vi "move2.vi"(8 "error in (no error)":errorcluster caption="错误输入（无错误）", 9 "动效风格":enum16{"风格一", "风格二", "风格三", "风格四"}(ring), 10 "In(T)/Out(F)":bool, 11 "Decor引用句柄":refnum<vi>) -> (0 "error out":errorcluster caption="错误输出")   [LabVIEW 2025, in "XButton.lvlib" / "button3.xctl"]
uses:
  button3.xctl
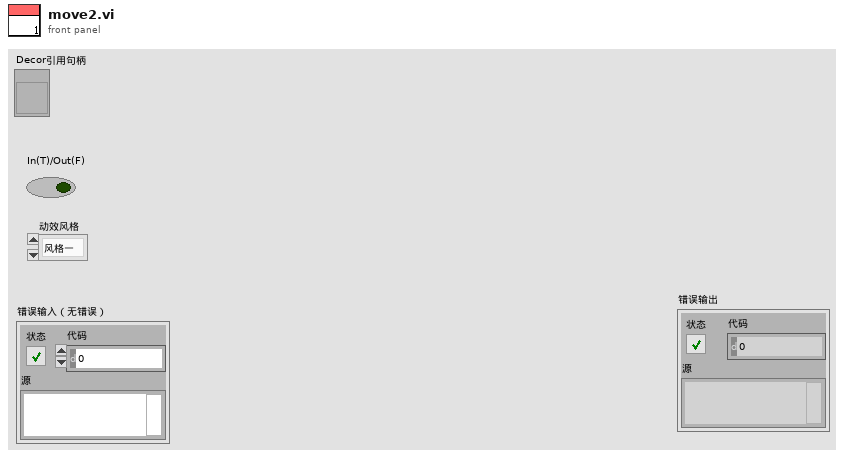
[diagram p1: front panel]
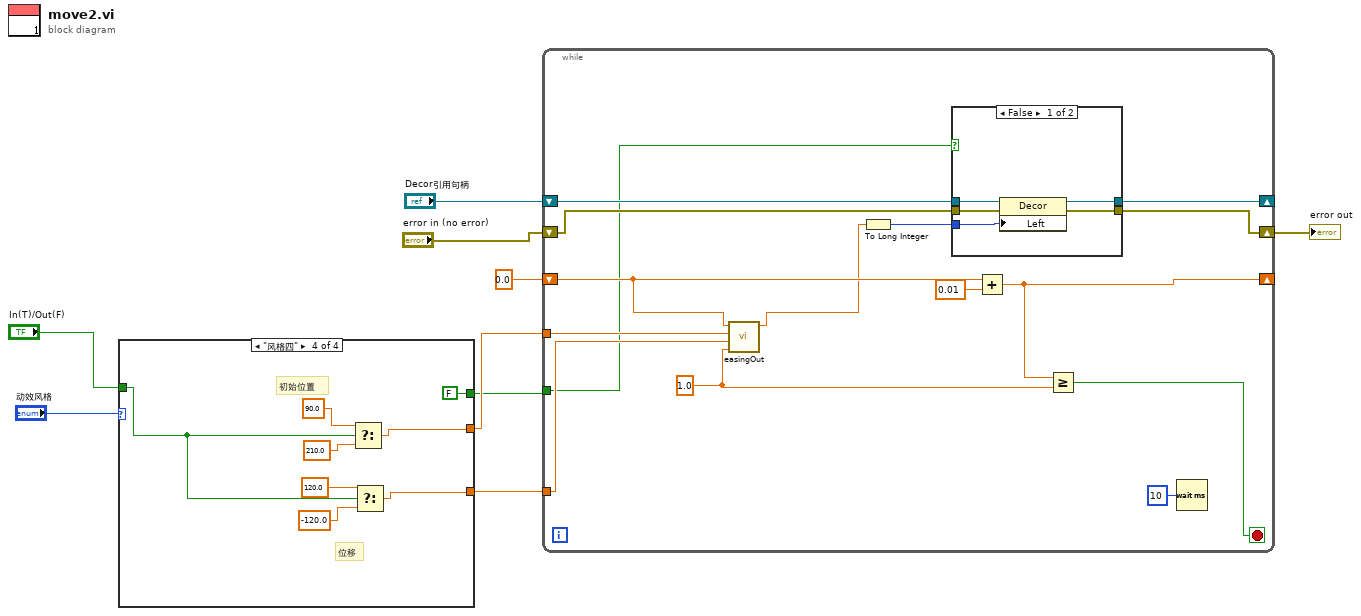
[diagram p0: block diagram]
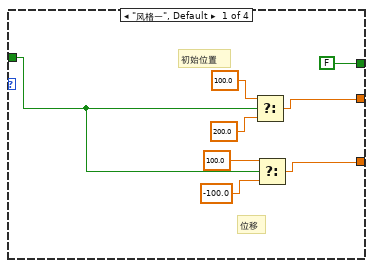
[diagram p2: hidden frame]
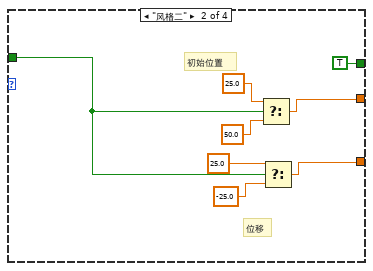
[diagram p3: hidden frame]
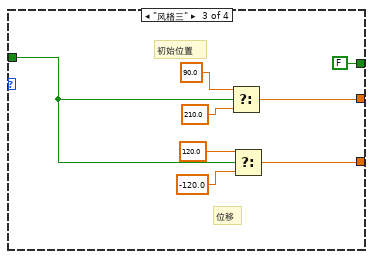
[diagram p4: hidden frame]
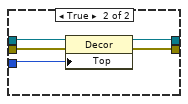
[diagram p5: hidden frame]
diagram:
  n1 = case shown="\"风格四\"" "动效风格" {
    tunnel: "In(T)/Out(F)" -> [w13 w21 w33 w35]
    tunnel: [w12 w20 w32 w37] -> w3
    tunnel: [w11 w19 w29 w36] -> w2
    tunnel: [FALSE TRUE FALSE FALSE] -> w1
    frame "风格一", Default {
      # "位移"
      # "初始位置"
      n2 = Select(t=100.0 ("b"), s=w13, f=200.0 ("b")) -> (s? t:f=w12:dbl)
      n3 = Select(t=100.0, s=w13, f=-100.0 ("c")) -> (s? t:f=w11:dbl)
    }
    frame "风格二" {
      # "位移"
      # "初始位置"
      n4 = Select(t=25.0 ("b"), s=w21, f=50.0 ("b")) -> (s? t:f=w20:dbl)
      n5 = Select(t=25.0, s=w21, f=-25.0 ("c")) -> (s? t:f=w19:dbl)
    }
    frame "风格三" {
      # "位移"
      # "初始位置"
      n6 = Select(t=90.0 ("b"), s=w33, f=210.0 ("b")) -> (s? t:f=w32:dbl)
      n7 = Select(t=120.0, s=w33, f=-120.0 ("c")) -> (s? t:f=w29:dbl)
    }
    frame "风格四" {
      # "位移"
      # "初始位置"
      n8 = Select(t=90.0 ("b"), s=w35, f=210.0 ("b")) -> (s? t:f=w37:dbl)
      n9 = Select(t=120.0, s=w35, f=-120.0 ("c")) -> (s? t:f=w36:dbl)
    }
  }
  n10 = while {
    shift-right: [w53] -> _
    shift-left: "Decor引用句柄" -> [w54]
    shift-right: [w46] -> _
    shift-left: 0.0 -> [w47]
    shift-right: [w51] -> w6
    shift-left: "error in (no error)" -> [w52]
    tunnel: w3 -> [w44]
    tunnel: w2 -> [w43]
    tunnel: w1 -> [w42]
    stop <- w48 stop-if-true
    w49 = 1.0 ("d")
    n11 = call "easingOut.vi"("d"=w49, "c"=w43, "b"=w44, "t"=w47) -> ("return"=w45:dbl)  [unwired: 7 in]
    n12 = To Long Integer(number=w45) -> (32bit integer=w50:i32)
    n13 = case shown="False" w42 {
      tunnel: w54 -> [w61 w66]
      tunnel: [w60 w65] -> w53
      tunnel: w52 -> [w59 w64]
      tunnel: [w58 w63] -> w51
      tunnel: w50 -> [w57 w62]
      frame False {
        n14 = property class="Decor"(reference=w61, error in=w59, "Left"=w57) -> (reference out=w60:refnum<vi>, error out=w58:errorcluster)
      }
      frame True {
        n15 = property class="Decor"(reference=w66, error in=w64, "Top"=w62) -> (reference out=w65:refnum<vi>, error out=w63:errorcluster)
      }
    }
    n16 = Add(x=w47, y=0.01) -> (x+y=w46:dbl)
    n17 = Greater Or Equal?(x=w46, y=w49) -> (x >= y?=w48:bool)
    n18 = Wait (ms)(milliseconds to wait=u32 10 ("等待时间（毫秒）")) -> ()  [unwired: 1 out]
  }
  "error out" <- w6
